vi "Initialize Resistor Interface.vi"(0 "Color Refn":T1, 1 "Selec Refn":T2, 3 "error in (no error)":errorcluster) -> (10 "error out":errorcluster)   [LabVIEW 2018, in "Front Panel Interface.lvlib"]
doc: "Initializes the resistor Front Panel interface to a known state.\n\nThe VI receives the clusters of <b>Selec Refn</b> and <b>Color Refn</b> corresponding to the six resistor band selectors and six resistor band ColorBox controls.\n\nIt sets the <b>Visible</b> property of all band selectors and ColorBox controls to <b>TRUE</b>, making all six resistor bands and their corresponding selectors visible.\n\nThis VI only establishes the initial Front Panel visibility state. It does not configure the interface according to the selected number of bands."
uses:
  Front Panel Interface.lvlib
  Resistor Controls/Selectors Refnums--cluster.ctl
  Resistor Controls/Digit--enum.ctl
  Resistor Controls/Multiplier--enum.ctl
  Resistor Controls/Tolerance--enum.ctl
  Resistor Controls/Temp Coefficient--enum.ctl
  Resistance Colors/Colors Refnums--cluster.ctl
  Resistor Controls/Resistance Controls.lvlib
  Resistance Colors/Resistance Colors.lvlib
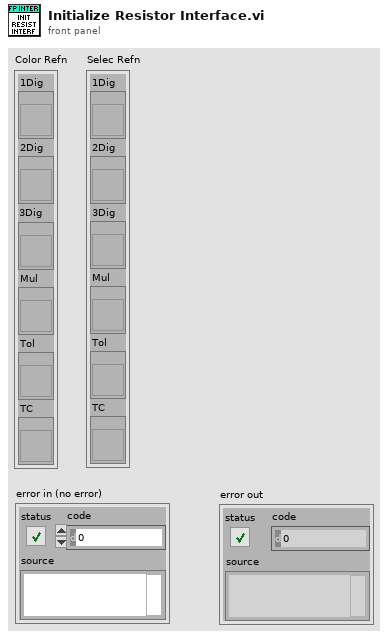
[diagram p1: front panel]
types:
  T1 = typedef "Resistance Colors.lvlib/Colors Refnums--cluster.ctl" = cluster{"1Dig":refnum<vi>, "2Dig":refnum<vi>, "3Dig":refnum<vi>, "Mul":refnum<vi>, "Tol":refnum<vi>, "TC":refnum<vi>}
  T2 = typedef "Resistance Controls.lvlib/Selectors Refnums--cluster.ctl" = cluster{"1Dig":refnum<vi>, "2Dig":refnum<vi>, "3Dig":refnum<vi>, "Mul":refnum<vi>, "Tol":refnum<vi>, "TC":refnum<vi>}
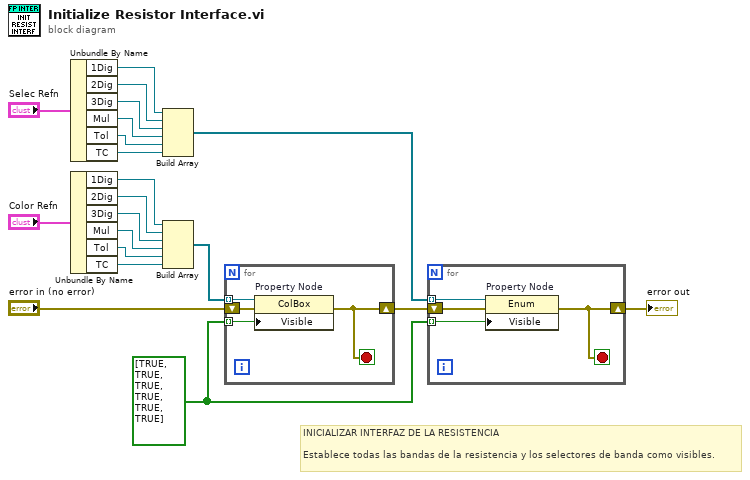
[diagram p0: block diagram]
diagram:
  w17 = bool[] [TRUE, TRUE, TRUE, TRUE, TRUE, TRUE]
  # "INICIALIZAR INTERFAZ DE LA RESISTENCIA\n\nEstablece todas las bandas de la resistencia y los selectores de banda como visibles."
  n1 = Unbundle By Name("Selec Refn") -> ("1Dig"=w15:refnum<vi>, "2Dig"=w14:refnum<vi>, "3Dig"=w13:refnum<vi>, "Mul"=w12:refnum<vi>, "Tol"=w11:refnum<vi>, "TC"=w10:refnum<vi>)
  n2 = Unbundle By Name("Color Refn") -> ("1Dig"=w6:refnum<vi>, "2Dig"=w5:refnum<vi>, "3Dig"=w4:refnum<vi>, "Mul"=w3:refnum<vi>, "Tol"=w2:refnum<vi>, "TC"=w1:refnum<vi>)
  n3 = Build Array(w15, w14, w13, w12, w11, w10) -> (w9:refnum<vi>[])
  n4 = Build Array(w6, w5, w4, w3, w2, w1) -> (w8:refnum<vi>[])
  n5 = for {
    tunnel: w8 -> [w24] mode=indexing
    tunnel: w17 -> [w23] mode=indexing
    shift-right: [w21] -> w19
    shift-left: "error in (no error)" -> [w22]
    stop <- w21 stop-if-true
    n6 = property on="Property Node" class="ColBox"(reference=w24, error in=w22, "Visible"=w23) -> (error out=w21:errorcluster)  [unwired: 1 out]
  }
  n7 = for {
    tunnel: w17 -> [w25] mode=indexing
    shift-right: [w27] -> w18
    shift-left: w19 -> [w28]
    tunnel: w9 -> [w26] mode=indexing
    stop <- w27 stop-if-true
    n8 = property on="Property Node" class="Enum"(reference=w26, error in=w28, "Visible"=w25) -> (error out=w27:errorcluster)  [unwired: 1 out]
  }
  "error out" <- w18
